vi "array and numeric.vi"() -> ()   [LabVIEW 2021]
panel:
  out "x-y":dbl[](array[numeric])
  in  "Numeric":dbl
  in  "Array":dbl[](array[numeric])
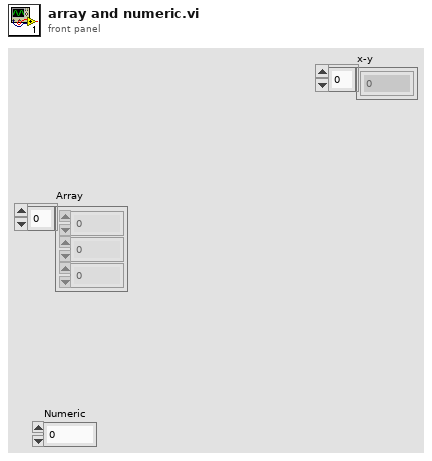
[diagram p1: front panel]
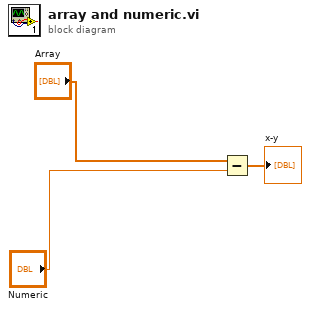
[diagram p0: block diagram]
diagram:
  n1 = Subtract(x="Array", y="Numeric") -> (x-y=→"x-y":dbl[])
